vi "Null Broadcast Events--constant.vi"() -> (3 "testCoordinator Broadcast Events":T1)   [LabVIEW 2026, in "testCoordinator.lvlib"]
doc: "Returns the broadcast events cluster with null references for defining the event types in a Register For Events function.\n_____\nBased on DQMH Dev Tools: Project Template 7.1.2.1547."
uses:
  testCoordinator.lvlib
  Broadcast Events--cluster.ctl
  Did Init Argument--cluster.ctl
  Status Updated Argument--cluster.ctl
  Error Reported Argument--cluster.ctl
  Do Something Argument--cluster.ctl
  Stop Argument--cluster.ctl
  Get Module Execution Status Argument--cluster.ctl
  Broadcast Available Tests Argument--cluster.ctl
  Refresh Test Procedure Indicator Argument--cluster.ctl
  Refresh Section Indicator Argument--cluster.ctl
  Refresh Instruction Indicator Argument--cluster.ctl
  Broadcast Test Scope Argument--cluster.ctl
  Broadcast Actual Test Procedure Section Argument--cluster.ctl
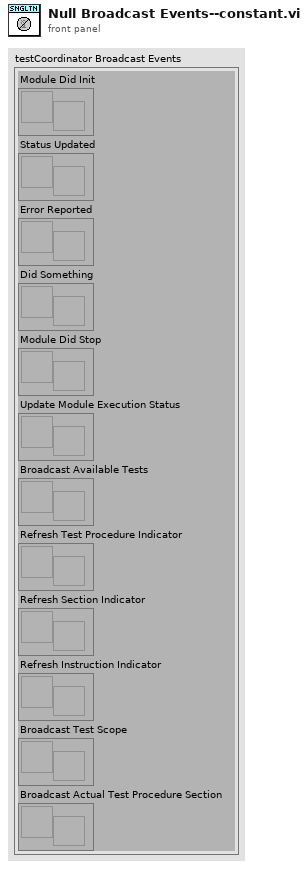
[diagram p1: front panel]
types:
  T1 = typedef "testCoordinator.lvlib/Broadcast Events--cluster.ctl" = cluster{"Module Did Init":refnum<user-event>, "Status Updated":refnum<user-event>, "Error Reported":refnum<user-event>, "Did Something":refnum<user-event>, "Module Did Stop":refnum<user-event>, "Update Module Execution Status":refnum<user-event>, "Broadcast Available Tests":refnum<user-event>, "Refresh Test Procedure Indicator":refnum<user-event>, "Refresh Section Indicator":refnum<user-event>, "Refresh Instruction Indicator":refnum<user-event>, "Broadcast Test Scope":refnum<user-event>, "Broadcast Actual Test Procedure Section":refnum<user-event>}
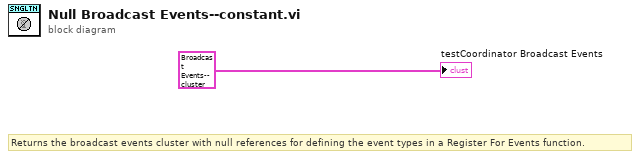
[diagram p0: block diagram]
diagram:
  # "Returns the broadcast events cluster with null references for defining the event types in a Register For Events function."
  "testCoordinator Broadcast Events" <- T1 {"Module Did Init"=refnum, "Status Updated"=refnum, "Error Reported"=refnum, "Did Something"=refnum, "Module Did Stop"=refnum, "Update Module Execution Status"=refnum, "Broadcast Available Tests"=refnum, "Refresh Test Procedure Indicator"=refnum, "Refresh Section Indicator"=refnum, "Refresh Instruction Indicator"=refnum, "Broadcast Test Scope"=refnum, "Broadcast Actual Test Procedure Section"=refnum} ("Broadcast Events")
